vi "Week 9 Tutorial.vi"() -> ()   [LabVIEW 2026]
panel:
  out "error out 2":errorcluster
  out "Port":i32
  out "Address":string="abc"
  in  "Send":bool
  out "error out":errorcluster
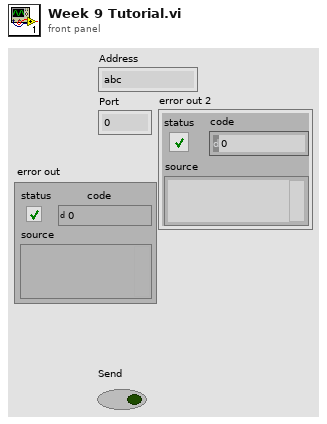
[diagram p1: front panel]
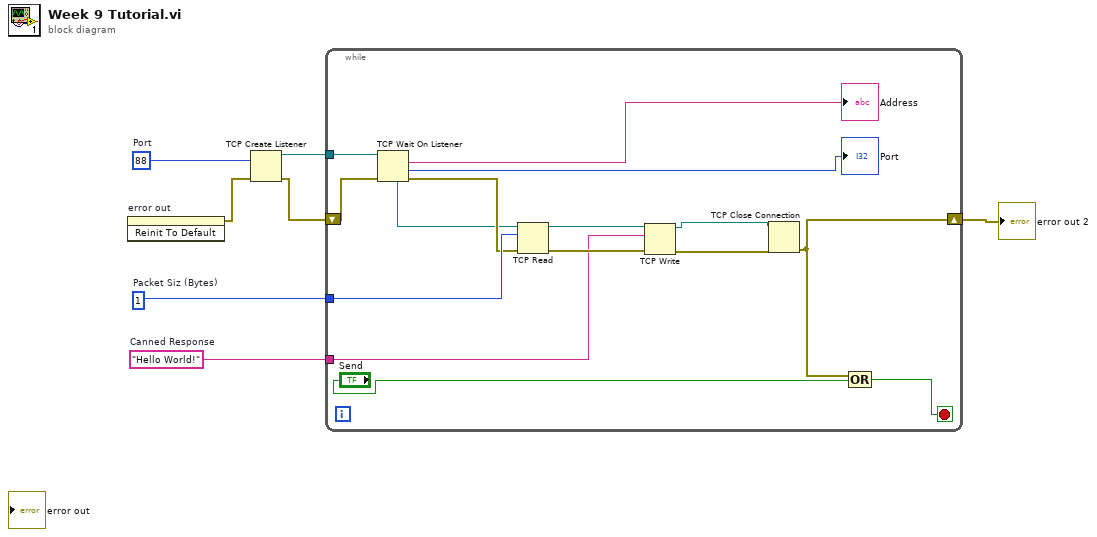
[diagram p0: block diagram]
diagram:
  w2 = "Hello World!"  # Canned Response
  w3 = 1  # Packet Siz (Bytes)
  w7 = 88  # Port
  n1 = invoke on="error out" class="Clust (strict)" method="Reinit To Default"() -> (error out=w5:errorcluster)  [unwired: 3 in, 2 out]
  n2 = TCP Create Listener(8:w5, 10:w7) -> (0:w4:errorcluster, 3:w6:refnum<k5>)  [unwired: 3 in, 1 out]
  n3 = while {
    tunnel: w6 -> [w18]
    tunnel: w3 -> [w19]
    tunnel: w2 -> [w20]
    shift-right: [w9] -> w1
    shift-left: w4 -> [w17]
    stop <- w10 stop-if-true
    n4 = TCP Wait On Listener(8:w17, 11:w18) -> (0:w14:errorcluster, 1:→"Port":u16, 2:→"Address":string, 4:w13:refnum<k5>)  [unwired: 2 in, 1 out]
    n5 = TCP Read(connection ID=w13, bytes to read=w19, error in (no error)=w14) -> (connection ID out=w12:refnum<k5>, error out=w22:errorcluster)  [unwired: 2 in, 1 out]
    n6 = TCP Write(connection ID=w12, data in=w20, error in (no error)=w22) -> (connection ID out=w8:refnum<k5>, error out=w21:errorcluster)  [unwired: 1 in, 1 out]
    n7 = TCP Close Connection(connection ID=w8, error in (no error)=w21) -> (error out=w9:errorcluster)  [unwired: 1 in, 1 out]
    n8 = Compound Arithmetic op=OR(w9, "Send") -> (w10:bool)
  }
  "error out 2" <- w1
